vi "Calculate Place points.vi"(8 "error in (no error)":errorcluster, 11 "Control in":refnum<class "Control.lvclass">) -> (0 "error out":errorcluster, 3 "Control out":refnum<class "Control.lvclass">)   [LabVIEW 2012, in "Control.lvclass"]
doc: "Calculates the position of the icon or text placement in the icon, based on the button orientation chosen."
uses:
  Control.lvclass
  Control.lvclass/Control.ctl
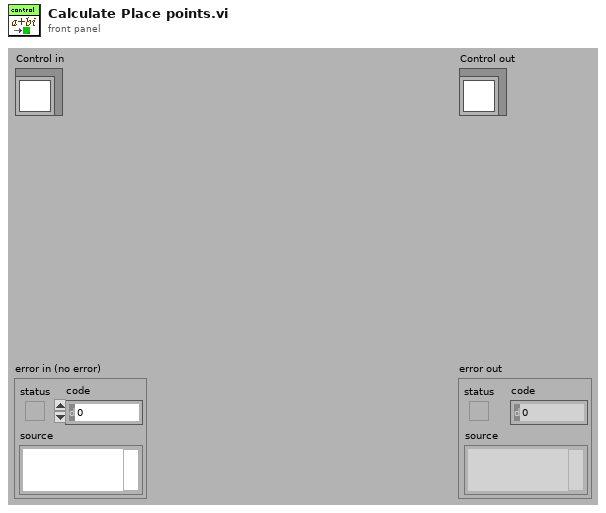
[diagram p1: front panel]
types:
  T1 = enum16{"User-specified Font", "Application Font", "System Font", "Dialog Font"}
  T2 = typedef "Control.lvclass/BX.Orientation__LCR _Modified.ctl" = u8
  T3 = typedef "Control.lvclass/_ui_tools_font.ctl" = cluster{"Font Name:":string, "Size":i16, "Strikeout?":bool, "Italic?":bool, "Underline?":bool, "Outline?":bool, "Shadow?":bool, "Bold?":bool}
  T4 = cluster{"left":i16, "top":i16, "right":i16, "bottom":i16}
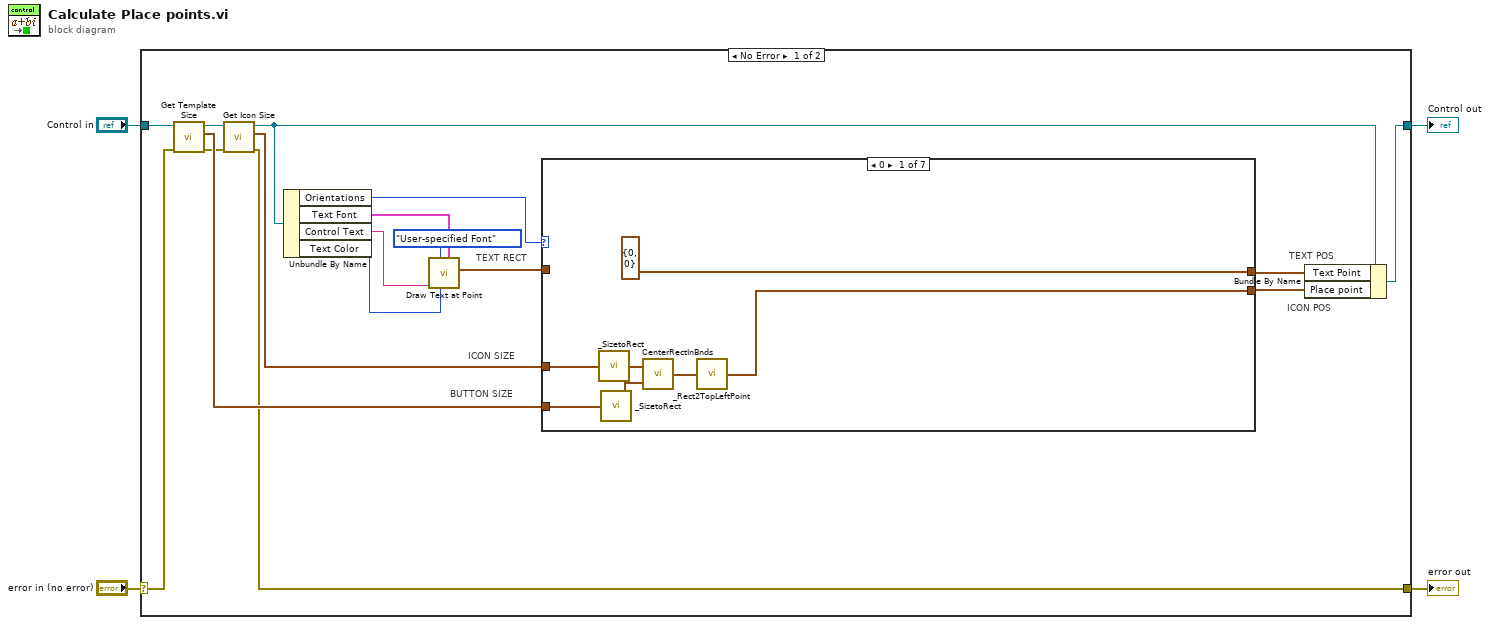
[diagram p0: block diagram]
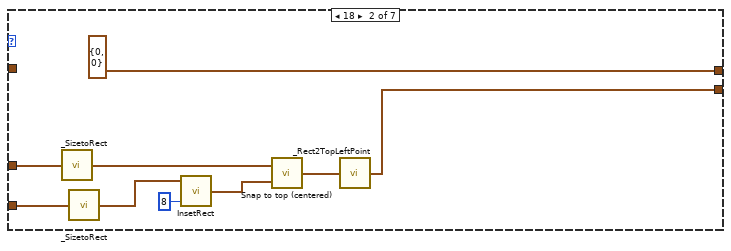
[diagram p2: hidden frame]
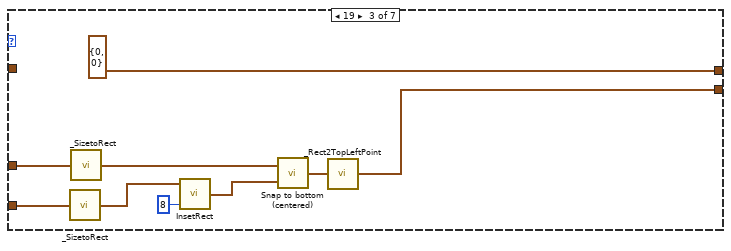
[diagram p3: hidden frame]
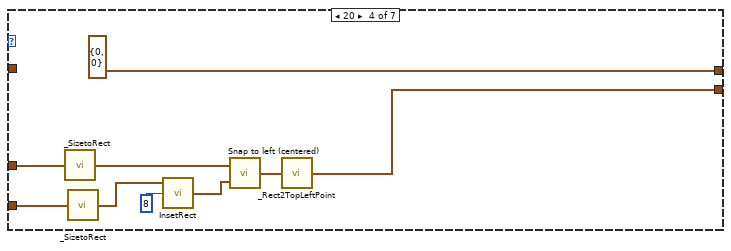
[diagram p4: hidden frame]
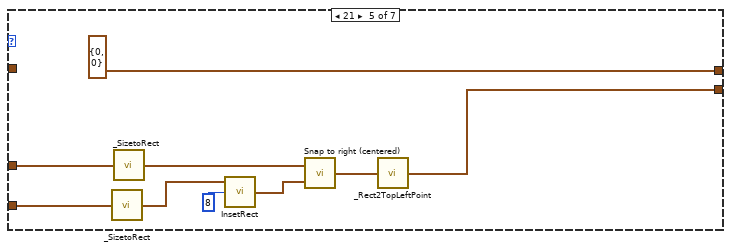
[diagram p5: hidden frame]
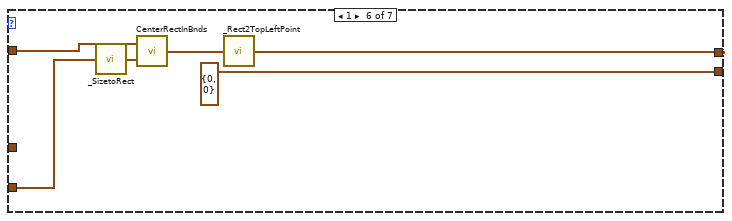
[diagram p6: hidden frame]
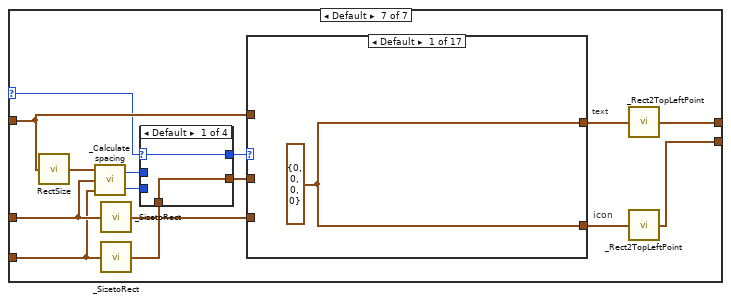
[diagram p7: hidden frame]
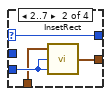
[diagram p8: hidden frame]
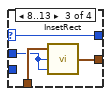
[diagram p9: hidden frame]
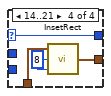
[diagram p10: hidden frame]
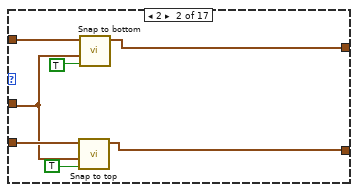
[diagram p11: hidden frame]
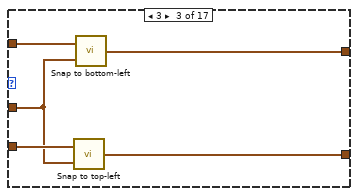
[diagram p12: hidden frame]
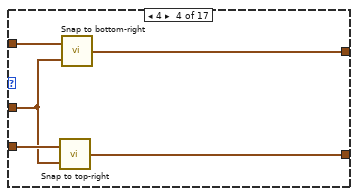
[diagram p13: hidden frame]
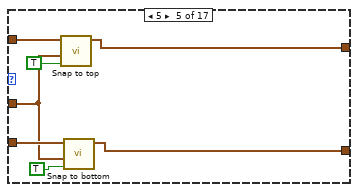
[diagram p14: hidden frame]
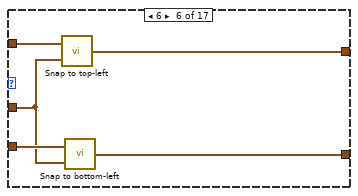
[diagram p15: hidden frame]
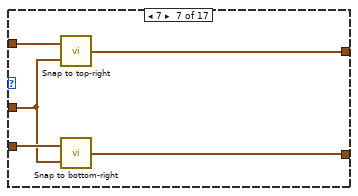
[diagram p16: hidden frame]
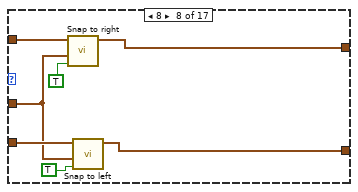
[diagram p17: hidden frame]
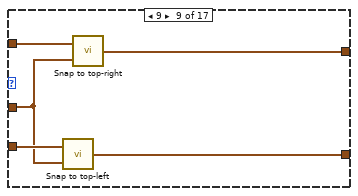
[diagram p18: hidden frame]
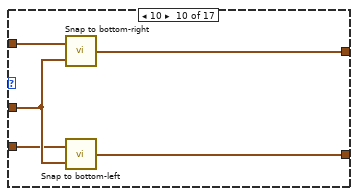
[diagram p19: hidden frame]
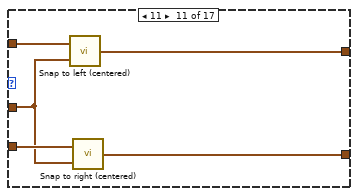
[diagram p20: hidden frame]
diagram:
  n1 = case shown="No Error" "error in (no error)" {
    selector: "error in (no error)" -> [w15 w203]
    tunnel: [w6 w203] -> w3
    tunnel: [w9 w202] -> w1
    tunnel: "Control in" -> [w14 w202]
    frame No Error {
      # "TEXT RECT"
      # "ICON SIZE"
      # "BUTTON SIZE"
      # "TEXT POS"
      # "ICON POS"
      n2 = call-dynamic "Get Template Size.vi"("error in (no error)"=w15, "Control in"=w14) -> ("error out"=w16:errorcluster, "Button Size"=w18:cluster{"Width":i32, "Height":i32}, "Control out"=w21:refnum<class "Control.lvclass">)  [unwired: 7 out]
      n3 = call-dynamic "Get Icon Size.vi"("error in (no error)"=w16, "Control in"=w21) -> ("error out"=w6:errorcluster, "Icon Size"=w19:cluster{"Width":i32, "Height":i32}, "Control out"=w10:refnum<class "Control.lvclass">)  [unwired: 7 out]
      n4 = Unbundle By Name(w10) -> ("Orientations"=w11:T2, "Text Font"=w12:T3, "Control Text"=w13:string, "Text Color"=w5:u32)
      n5 = call <vilib>:"Draw Text at Point.vi"("[user-specified font]"=w12, "text color(black)"=w5, "desired font(Application)"=T1."User-specified Font", "text"=w13) -> ("text rect"=w17:T4)  [unwired: 5 in, 2 out]
      n6 = case shown="0" w11 {
        selector: w11 -> [_ _ _ _ _ _ w83]
        tunnel: [cluster{"x":i32, "y":i32} {"x"=0, "y"=0} ("Point") cluster{"x":i32, "y":i32} {"x"=0, "y"=0} ("Point") cluster{"x":i32, "y":i32} {"x"=0, "y"=0} ("Point") cluster{"x":i32, "y":i32} {"x"=0, "y"=0} ("Point") cluster{"x":i32, "y":i32} {"x"=0, "y"=0} ("Point") w65 w71] -> w8
        tunnel: [w22 w32 w41 w50 w57 cluster{"x":i32, "y":i32} {"x"=0, "y"=0} ("Point") w72] -> w7
        tunnel: w18 -> [w26 w33 w43 w48 w61 w68 w77]
        tunnel: w17 -> [_ _ _ _ _ w70 w85]
        tunnel: w19 -> [w24 w35 w44 w52 w62 _ w78]
        frame 0 {
          n7 = call "_SizetoRect.vi"("size"=w24) -> ("bounds"=w25:T4)  [unwired: 4 out]
          n8 = call "_SizetoRect.vi"("size"=w26) -> ("bounds"=w27:T4)  [unwired: 4 out]
          n9 = call <vilib>:"CenterRectInBnds.vi"("bounds"=w27, "rect"=w25) -> ("centered rect"=w23:T4)
          n10 = call "_Rect2TopLeftPoint.vi"("bounds"=w23) -> ("TopLeft point"=w22:cluster{"x":i32, "y":i32})  [unwired: 4 out]
        }
        frame 18 {
          n11 = call "_SizetoRect.vi"("size"=w35) -> ("bounds"=w31:T4)  [unwired: 4 out]
          n12 = call "_SizetoRect.vi"("size"=w33) -> ("bounds"=w34:T4)  [unwired: 4 out]
          n13 = call <vilib>:"InsetRect.vi"("dv"=i16 8 ("dh"), "rect"=w34) -> ("inset rect"=w30:T4)  [unwired: 1 in]
          n14 = call "Snap to top (centered).vi"("Large Rect"=w30, "Small Rect"=w31) -> ("Snapped to top center"=w29:T4)
          n15 = call "_Rect2TopLeftPoint.vi"("bounds"=w29) -> ("TopLeft point"=w32:cluster{"x":i32, "y":i32})  [unwired: 4 out]
        }
        frame 19 {
          n16 = call "_SizetoRect.vi"("size"=w43) -> ("bounds"=w42:T4)  [unwired: 4 out]
          n17 = call "_SizetoRect.vi"("size"=w44) -> ("bounds"=w40:T4)  [unwired: 4 out]
          n18 = call <vilib>:"InsetRect.vi"("dv"=i16 8 ("dh"), "rect"=w42) -> ("inset rect"=w39:T4)  [unwired: 1 in]
          n19 = call "Snap to bottom (centered).vi"("Large Rect"=w39, "Small Rect"=w40) -> ("Snapped to bottom center"=w38:T4)
          n20 = call "_Rect2TopLeftPoint.vi"("bounds"=w38) -> ("TopLeft point"=w41:cluster{"x":i32, "y":i32})  [unwired: 4 out]
        }
        frame 20 {
          n21 = call "_SizetoRect.vi"("size"=w52) -> ("bounds"=w53:T4)  [unwired: 4 out]
          n22 = call "_SizetoRect.vi"("size"=w48) -> ("bounds"=w47:T4)  [unwired: 4 out]
          n23 = call <vilib>:"InsetRect.vi"("dh"=i16 8, "rect"=w47) -> ("inset rect"=w49:T4)  [unwired: 1 in]
          n24 = call "Snap to left (centered).vi"("Large Rect"=w49, "Small Rect"=w53) -> ("Snapped to left center"=w51:T4)
          n25 = call "_Rect2TopLeftPoint.vi"("bounds"=w51) -> ("TopLeft point"=w50:cluster{"x":i32, "y":i32})  [unwired: 4 out]
        }
        frame 21 {
          n26 = call "_SizetoRect.vi"("size"=w61) -> ("bounds"=w60:T4)  [unwired: 4 out]
          n27 = call "_SizetoRect.vi"("size"=w62) -> ("bounds"=w59:T4)  [unwired: 4 out]
          n28 = call <vilib>:"InsetRect.vi"("dh"=i16 8, "rect"=w60) -> ("inset rect"=w58:T4)  [unwired: 1 in]
          n29 = call "Snap to right (centered).vi"("Large Rect"=w58, "Small Rect"=w59) -> ("Snapped to right center"=w56:T4)
          n30 = call "_Rect2TopLeftPoint.vi"("bounds"=w56) -> ("TopLeft point"=w57:cluster{"x":i32, "y":i32})  [unwired: 4 out]
        }
        frame 1 {
          n31 = call "_SizetoRect.vi"("size"=w68) -> ("bounds"=w67:T4)  [unwired: 4 out]
          n32 = call <vilib>:"CenterRectInBnds.vi"("bounds"=w67, "rect"=w70) -> ("centered rect"=w66:T4)
          n33 = call "_Rect2TopLeftPoint.vi"("bounds"=w66) -> ("TopLeft point"=w65:cluster{"x":i32, "y":i32})  [unwired: 4 out]
        }
        frame Default {
          # "icon"
          # "text"
          n34 = call <vilib>:"RectSize.vi"("rect"=w85) -> ("point"=w79:cluster{"x":i16, "y":i16})
          n35 = call "_Calculate spacing.vi"("Button Size"=w77, "Icon Size"=w78, "Text Size"=w79) -> ("Vert. spacing"=w75:i32, "Horiz. spacing"=w76:i32)
          n36 = call "_SizetoRect.vi"("size"=w78) -> ("bounds"=w80:T4)  [unwired: 4 out]
          n37 = call "_SizetoRect.vi"("size"=w77) -> ("bounds"=w81:T4)  [unwired: 4 out]
          n38 = case shown="Default" w83 {
            selector: w83 -> [w86 w88 w92 w97]
            tunnel: w75 -> [_ w91 _ _]
            tunnel: [w87 w90 w95 w99] -> w84
            tunnel: w81 -> [w87 w89 w94 w98]
            tunnel: w76 -> [_ _ w93 _]
            tunnel: [w86 w88 w92 w97] -> w82
            frame Default {
            }
            frame 2..7 {
              n39 = call <vilib>:"InsetRect.vi"("dv"=w91, "dh"=w91, "rect"=w89) -> ("inset rect"=w90:T4)
            }
            frame 8..13 {
              n40 = call <vilib>:"InsetRect.vi"("dv"=w93, "dh"=w93, "rect"=w94) -> ("inset rect"=w95:T4)
            }
            frame 14..21 {
              w96 = i16 8 ("dh")
              n41 = call <vilib>:"InsetRect.vi"("dv"=w96, "dh"=w96, "rect"=w98) -> ("inset rect"=w99:T4)
            }
          }
          n42 = case shown="Default" w82 {
            tunnel: w80 -> [_ w107 w110 w117 w121 w127 w134 w141 w146 w148 w154 w160 w163 w178 w184 w196 w198]
            tunnel: [w100 w105 w108 w116 w119 w125 w131 w139 w145 w147 w152 w161 w164 w173 w183 w195 w199] -> w73
            tunnel: w85 -> [_ w104 w112 w115 w124 w129 w133 w138 w144 w150 w156 w159 w165 w177 w182 w194 w201]
            tunnel: w84 -> [_ w102 w109 w114 w120 w126 w132 w137 w143 w151 w153 w158 w162 w176 w181 w193 w197]
            tunnel: [w100 w103 w111 w113 w122 w128 w130 w135 w142 w149 w155 w157 w166 w174 w191 w192 w200] -> w74
            frame Default {
              w100 = T4 {"left"=0, "top"=0, "right"=0, "bottom"=0} ("Snapped to bottom left")
            }
            frame 2 {
              n43 = call "Snap to top.vi"("centered? (F)"=TRUE, "Fixed Rect"=w102, "Rect"=w107) -> ("Snapped to top"=w105:T4)  [unwired: 8 out]
              n44 = call "Snap to bottom.vi"("centered? (F)"=TRUE, "Fixed Rect"=w102, "Rect"=w104) -> ("Snapped to bottom"=w103:T4)  [unwired: 8 out]
            }
            frame 3 {
              n45 = call "Snap to top-left.vi"("Fixed Rect"=w109, "Rect"=w110) -> ("Snapped to top left"=w108:T4)
              n46 = call "Snap to bottom-left.vi"("Fixed Rect"=w109, "Rect"=w112) -> ("Snapped to bottom left"=w111:T4)
            }
            frame 4 {
              n47 = call "Snap to top-right.vi"("Fixed Rect"=w114, "Rect"=w117) -> ("Snapped to top left"=w116:T4)
              n48 = call "Snap to bottom-right.vi"("Fixed Rect"=w114, "Rect"=w115) -> ("Snapped to bottom right"=w113:T4)
            }
            frame 5 {
              n49 = call "Snap to top.vi"("centered? (F)"=TRUE, "Fixed Rect"=w120, "Rect"=w124) -> ("Snapped to top"=w122:T4)  [unwired: 8 out]
              n50 = call "Snap to bottom.vi"("centered? (F)"=TRUE, "Fixed Rect"=w120, "Rect"=w121) -> ("Snapped to bottom"=w119:T4)  [unwired: 8 out]
            }
            frame 6 {
              n51 = call "Snap to top-left.vi"("Fixed Rect"=w126, "Rect"=w129) -> ("Snapped to top left"=w128:T4)
              n52 = call "Snap to bottom-left.vi"("Fixed Rect"=w126, "Rect"=w127) -> ("Snapped to bottom left"=w125:T4)
            }
            frame 7 {
              n53 = call "Snap to top-right.vi"("Fixed Rect"=w132, "Rect"=w133) -> ("Snapped to top left"=w130:T4)
              n54 = call "Snap to bottom-right.vi"("Fixed Rect"=w132, "Rect"=w134) -> ("Snapped to bottom right"=w131:T4)
            }
            frame 8 {
              n55 = call "Snap to right.vi"("centered? (F)"=TRUE, "Fixed Rect"=w137, "Rect"=w138) -> ("Snapped to right"=w135:T4)  [unwired: 8 out]
              n56 = call "Snap to left.vi"("centered? (F)"=TRUE, "Fixed Rect"=w137, "Rect"=w141) -> ("Snapped to left"=w139:T4)  [unwired: 8 out]
            }
            frame 9 {
              n57 = call "Snap to top-left.vi"("Fixed Rect"=w143, "Rect"=w146) -> ("Snapped to top left"=w145:T4)
              n58 = call "Snap to top-right.vi"("Fixed Rect"=w143, "Rect"=w144) -> ("Snapped to top left"=w142:T4)
            }
            frame 10 {
              n59 = call "Snap to bottom-right.vi"("Fixed Rect"=w151, "Rect"=w150) -> ("Snapped to bottom right"=w149:T4)
              n60 = call "Snap to bottom-left.vi"("Fixed Rect"=w151, "Rect"=w148) -> ("Snapped to bottom left"=w147:T4)
            }
            frame 11 {
              n61 = call "Snap to left (centered).vi"("Large Rect"=w153, "Small Rect"=w156) -> ("Snapped to left center"=w155:T4)
              n62 = call "Snap to right (centered).vi"("Large Rect"=w153, "Small Rect"=w154) -> ("Snapped to right center"=w152:T4)
            }
            frame 12 {
              n63 = call "Snap to top-right.vi"("Fixed Rect"=w158, "Rect"=w160) -> ("Snapped to top left"=w161:T4)
              n64 = call "Snap to top-left.vi"("Fixed Rect"=w158, "Rect"=w159) -> ("Snapped to top left"=w157:T4)
            }
            frame 13 {
              n65 = call "Snap to bottom-left.vi"("Fixed Rect"=w162, "Rect"=w165) -> ("Snapped to bottom left"=w166:T4)
              n66 = call "Snap to bottom-right.vi"("Fixed Rect"=w162, "Rect"=w163) -> ("Snapped to bottom right"=w164:T4)
            }
            frame 14 {
              n67 = call "Snap to left (centered).vi"("Large Rect"=w176, "Small Rect"=w177) -> ("Snapped to left center"=w175:T4)
              n68 = call "Snap to left (centered).vi"("Large Rect"=w176, "Small Rect"=w178) -> ("Snapped to left center"=w173:T4)
              n69 = call <vilib>:"RectSize.vi"("rect"=w173) -> ("point"=w172:cluster{"x":i16, "y":i16})
              n70 = Unbundle By Name(w172) -> ("x"=w171:i16)
              n71 = Add(x=w171, y=i16 12) -> (x+y=w167:i16)
              n72 = Bundle By Name(cluster=cluster{"x":i16, "y":i16} {"x"=0, "y"=0} ("point"), "x"=w167) -> (w168:cluster{"x":i16, "y":i16})
              n73 = call <vilib>:"POffsetRect.vi"("rect"=w175, "point"=w168) -> ("offset rect"=w174:T4)
            }
            frame 17 {
              n74 = call "Snap to right (centered).vi"("Large Rect"=w181, "Small Rect"=w182) -> ("Snapped to right center"=w180:T4)
              n75 = call "Snap to right (centered).vi"("Large Rect"=w181, "Small Rect"=w184) -> ("Snapped to right center"=w183:T4)
              n76 = call <vilib>:"RectSize.vi"("rect"=w183) -> ("point"=w190:cluster{"x":i16, "y":i16})
              n77 = Unbundle By Name(w190) -> ("x"=w189:i16)
              n78 = Add(x=w189, y=i16 12) -> (x+y=w185:i16)
              n79 = Negate(x=w185) -> (-x=w179:i16)
              n80 = Bundle By Name(cluster=cluster{"x":i16, "y":i16} {"x"=0, "y"=0} ("point"), "x"=w179) -> (w186:cluster{"x":i16, "y":i16})
              n81 = call <vilib>:"POffsetRect.vi"("rect"=w180, "point"=w186) -> ("offset rect"=w191:T4)
            }
            frame 15 {
              n82 = call "Snap to left (centered).vi"("Large Rect"=w193, "Small Rect"=w196) -> ("Snapped to left center"=w195:T4)
              n83 = call "Snap to right (centered).vi"("Large Rect"=w193, "Small Rect"=w194) -> ("Snapped to right center"=w192:T4)
            }
            frame 16 {
              n84 = call "Snap to left (centered).vi"("Large Rect"=w197, "Small Rect"=w201) -> ("Snapped to left center"=w200:T4)
              n85 = call "Snap to right (centered).vi"("Large Rect"=w197, "Small Rect"=w198) -> ("Snapped to right center"=w199:T4)
            }
          }
          n86 = call "_Rect2TopLeftPoint.vi"("bounds"=w74) -> ("TopLeft point"=w71:cluster{"x":i32, "y":i32})  [unwired: 4 out]
          n87 = call "_Rect2TopLeftPoint.vi"("bounds"=w73) -> ("TopLeft point"=w72:cluster{"x":i32, "y":i32})  [unwired: 4 out]
        }
      }
      n88 = Bundle By Name(cluster=w10, "Text Point"=w8, "Place point"=w7) -> (w9:refnum<class "Control.lvclass">)
    }
    frame Error {
    }
  }
  "error out" <- w3
  "Control out" <- w1
